vi "JS Chart.vi"() -> ()   [LabVIEW 2020]
uses:
  C:/Users/Simon/Documents/GitHub/LV-WebView2/Source/Libs/Microsoft.Web.WebView2.WinForms.dll
  Libs/Microsoft.Web.WebView2.WinForms.dll
  Webview2 Lib/WebView2 Control Object/Register Events.vi
  Webview2 Lib/WebView2 Control Object/Paths.ctl
  Webview2 Lib/WebView2 Control Object/WebView2 Control.lvclass
panel:
  out "time":timestamp
  out "Y":dbl
  out "Timed Out":bool
  in  "Chart Label":string
  in  "Stop":bool
  in  "WebView2":refnum<k24>(container)
  # "Clicked Coords"
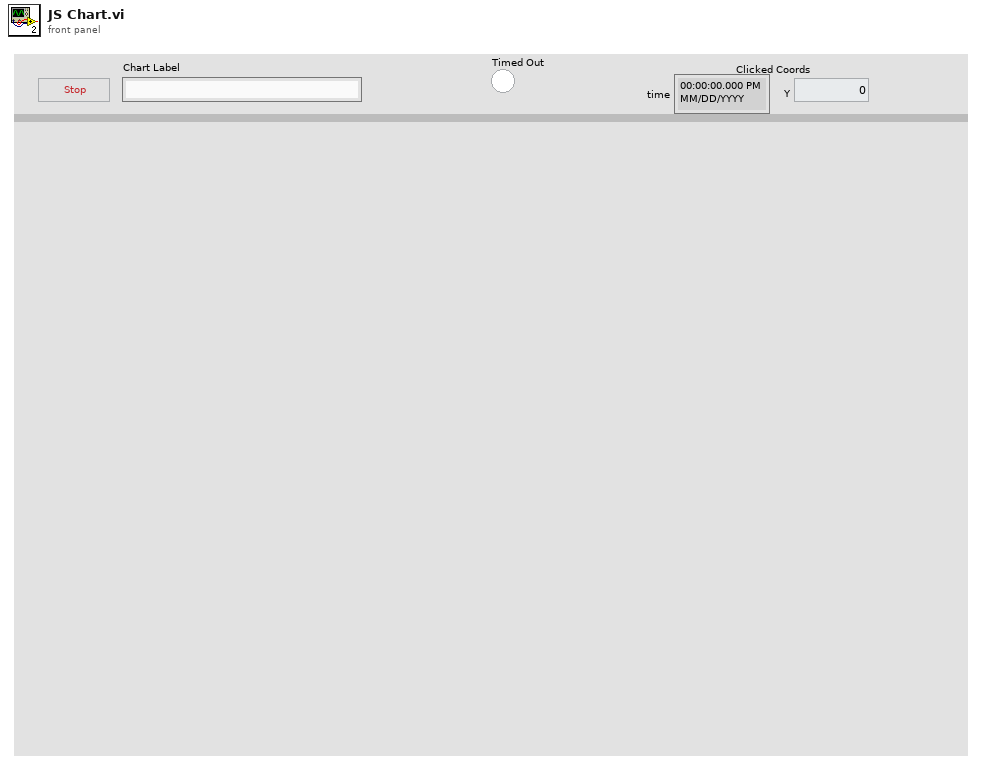
[diagram p1: front panel]
types:
  T1 = typedef "WebView2.lvlib/WebView2 Control.lvclass/Paths.ctl" = cluster{"Webview2 Native":path, "Edge Application":path, "User Data":path}
  T2 = typedef "WebView2.lvlib/WebView2 Control.lvclass/Events.ctl" = cluster{"Navigation Complete Event":refnum<user-event>, "Source Changed Event":refnum<user-event>, "Document Title Changed Event":refnum<user-event>, "Status Bar Text Changed":refnum<user-event>, "Web Message Received":refnum<user-event>, "Window Close Requested":refnum<user-event>, "DOM Loaded":refnum<user-event>, "Navigation Started Event":refnum<user-event>}
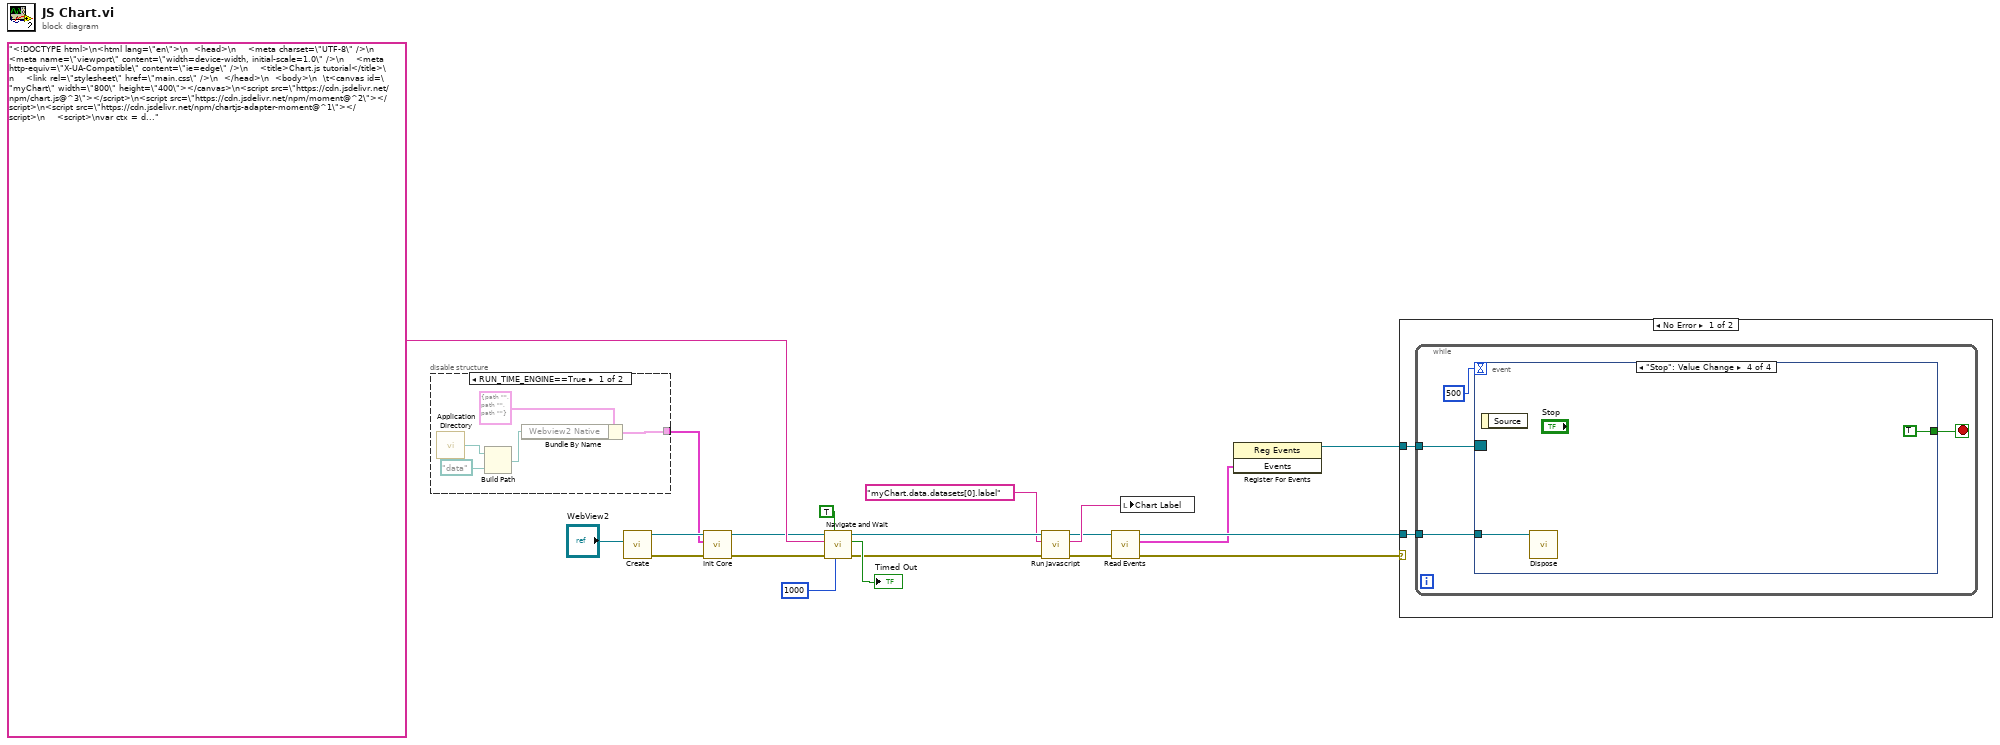
[diagram p0: block diagram]
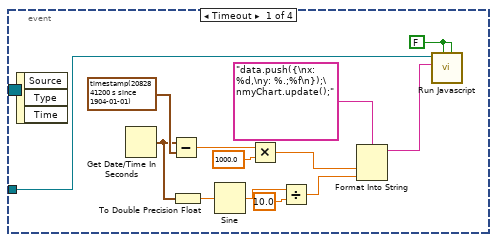
[diagram p2: hidden frame]
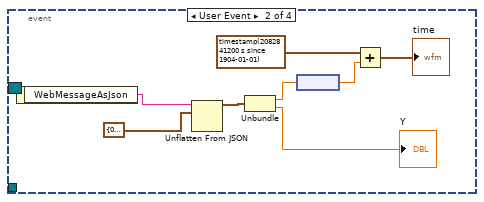
[diagram p3: hidden frame]
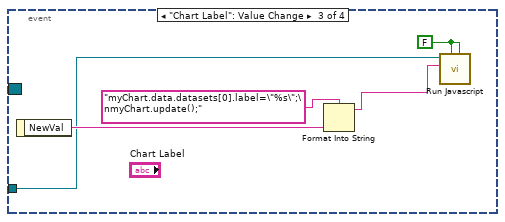
[diagram p4: hidden frame]
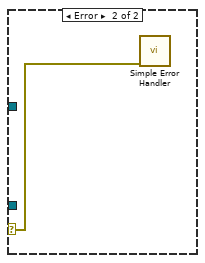
[diagram p5: hidden frame]
diagram:
  n1 = disable-structure shown="RUN_TIME_ENGINE==True" {
    disable-tunnel: [w21 _] -> w14
    frame condition #0 {
      n2 = call <vilib>:"Application Directory.vi"() -> ("Application Directory"=w24:path)
      n3 = Build Path(base path=w24, name or relative path=path "data") -> (appended path=w22:path)
      n4 = Bundle By Name(cluster=T1 {"Webview2 Native"=path "", "Edge Application"=path "", "User Data"=path ""} ("Paths"), "Webview2 Native"=w22) -> (w21:T1)
    }
    frame condition #1 (active) {
    }
  }
  n5 = call "Create.vi"("WebView2 Control"="WebView2") -> ("error out"=w13:errorcluster, "WebView2 Control out"=w15:refnum<class "WebView2 Control.lvclass">)  [unwired: 9 in]
  n6 = call "Init Core.vi"("error in (no error)"=w13, "Path Overrides (Empty=Default)"=w14, "WebView2 Control in"=w15) -> ("error out"=w17:errorcluster, "WebView2 Control out"=w18:refnum<class "WebView2 Control.lvclass">)  [unwired: 7 in]
  n7 = call "Navigate and Wait.vi"("Timeout (Inf)"=1000, "html Source (URL)"=TRUE, "error in (no error)"=w17, "Source"="<!DOCTYPE html>\n<html lang=\"en\">\n  <head>\n    <meta charset=\"UTF-8\" />\n    <meta name=\"viewport\" content=\"width=device-width, initial-scale=1.0\" />\n    <meta http-equiv=\"X-UA-Compatible\" content=\"ie=edge\" />\n    <title>Chart.js tutorial</title>\n    <link rel=\"stylesheet\" href=\"main.css\" />\n  </head>\n  <body>\n  \t<canvas id=\"myChart\" width=\"800\" height=\"400\"></canvas>\n<script src=\"https://cdn.jsdelivr.net/npm/chart.js@^3\"></script>\n<script src=\"https://cdn.jsdelivr.net/npm/moment@^2\"></script>\n<script src=\"https://cdn.jsdelivr.net/npm/chartjs-adapter-moment@^1\"></script>\n    <script>\nvar ctx = document.getElementById(\"myChart\");\n\nvar data = []\n\nvar myChart = new Chart(ctx, {\n type: \"line\",\n options: {\n        scales: {\n                x: {\n                        type: 'time'\n                }\n        },\n        onClick: (e) => {\n            const canvasPosition = Chart.helpers.getRelativePosition(e, myChart);\n\n            const dataX = myChart.scales.x.getValueForPixel(canvasPosition.x);\n            const dataY = myChart.scales.y.getValueForPixel(canvasPosition.y);\n            window.chrome.webview.postMessage({'X':dataX,'Y':dataY});\n        }\n },\n data: {\n    datasets: [\n    {\n\t\tlabel: \"Data\",\n        data: data,\n        backgroundColor: \"rgba(255, 99, 132, 0.2)\",\n        borderColor: \"rgba(255, 99, 132, 1)\",\n        borderWidth: 1\n    }\n    ]\n }\n});\nwindow.chrome.webview.postMessage(\"test\");\n\t</script>\n  </body>\n</html>\n", "WebView2 Control in"=w18) -> ("error out"=w2:errorcluster, "Timed Out"=→"Timed Out":bool, "WebView2 Control out"=w19:refnum<class "WebView2 Control.lvclass">)  [unwired: 4 in]
  n8 = call "Run Javascript.vi"("error in (no error)"=w2, "javaScript"="myChart.data.datasets[0].label", "WebView2 Control in"=w19) -> ("error out"=w1:errorcluster, "Result"=w8:string, "WebView2 Control out"=w6:refnum<class "WebView2 Control.lvclass">)  [unwired: 6 in]
  n9 = call "Read Events.vi"("error in (no error)"=w1, "WebView2 Control in"=w6) -> ("error out"=w7:errorcluster, "Events"=w4:T2, "WebView2 Control out"=w5:refnum<class "WebView2 Control.lvclass">)  [unwired: 7 in]
  n10 = local write "Chart Label"(w8) -> ()
  n11 = register-events(w4) -> (reference out=w3:refnum<event-registration>)  [unwired: 2 in, 1 out]
  n12 = case shown="No Error" w7 {
    selector: w7 -> [_ w60]
    tunnel: w5 -> [w27 _]
    tunnel: w3 -> [w26 _]
    frame No Error {
      n13 = while {
        tunnel: w27 -> [w29]
        tunnel: w26 -> [w28]
        stop <- w30 stop-if-true
        n14 = event shown="[3] \"Stop\": Value Change" {
          selector: w28 -> [_ _ _ _]
          dyn-events: _ -> [_ _ _ _]
          timeout: 500 -> [_ _ _ _]
          tunnel: [_ _ _ TRUE] -> w30
          tunnel: w29 -> [w34 _ w55 w58]
          event Timeout {
            w32 = FALSE ("Decode Result")
            n15 = event-data() -> ()  [unwired: 1 in, 3 out]
            n16 = Get Date/Time In Seconds() -> (seconds since 1Jan1904=w36:timestamp)
            n17 = Subtract(x=w36, y=timestamp(2082841200 s since 1904-01-01) ("current time")) -> (x-y=w38:dbl)
            n18 = To Double Precision Float(number=w36) -> (double precision float=w43:dbl)
            n19 = Sine(x=w43) -> (sin(x)=w42:dbl)
            n20 = Multiply(x=w38, y=1000.0) -> (x*y=w35:dbl)
            n21 = Divide(x=w42, y=10.0) -> (x/y=w41:dbl)
            n22 = Format Into String(format string="data.push({\nx: %d,\ny: %.;%f\n});\nmyChart.update();" ("javaScript"), w35, w41) -> (resulting string=w33:string)  [unwired: 2 in, 1 out]
            n23 = call "Run Javascript.vi"("Decode Result (T)"=w32, "Fetch Result (T)"=w32, "javaScript"=w33, "WebView2 Control in"=w34) -> ()  [unwired: 5 in, 3 out]
          }
          event User Event {
            n24 = event-data() -> ("WebMessageAsJson"=w52:string)  [unwired: 1 in]
            n25 = Unflatten From JSON(JSON string=w52, type and defaults=cluster{"X":dbl, "Y":dbl} {"X"=0.0, "Y"=0.0}) -> (value=w50:cluster{"X":dbl, "Y":dbl})  [unwired: 5 in, 1 out]
            n26 = Unbundle(w50) -> ("X"=w46:dbl, "Y"=→"Y":dbl)
            n27 = node(w46) -> (w45:dbl[unit])
            n28 = Add(x=timestamp(2082841200 s since 1904-01-01), y=w45) -> (x+y=→"time":timestamp)
          }
          event "Chart Label": Value Change {
            w53 = FALSE ("Decode Result")
            n29 = event-data() -> ("NewVal"=w56:string)  [unwired: 1 in]
            n30 = Format Into String(format string="myChart.data.datasets[0].label=\"%s\";\nmyChart.update();" ("javaScript"), w56) -> (resulting string=w54:string)  [unwired: 2 in, 1 out]
            n31 = call "Run Javascript.vi"("Decode Result (T)"=w53, "Fetch Result (T)"=w53, "javaScript"=w54, "WebView2 Control in"=w55) -> ()  [unwired: 5 in, 3 out]
          }
          event "Stop": Value Change {
            n32 = event-data() -> ()  [unwired: 1 in, 1 out]
            n33 = call "Dispose.vi"("WebView2 Control in"=w58) -> ()  [unwired: 10 in, 1 out]
          }
        }
      }
    }
    frame Error {
      n34 = call <vilib>:"Simple Error Handler.vi"("error in (no error)"=w60) -> ()  [unwired: 4 in, 5 out]
    }
  }
